vi "libssh2_userauth_publickey_fromfile_ex.vi"(5 "private key":path, 7 "public key":path, 8 "error in (no error)":errorcluster, 9 "passphrase":string, 10 "username":string, 11 "session":T1) -> (0 "error out":errorcluster)   [LabVIEW 2017, in "libssh2.lvlib"]
doc: "Authenticate a session using a private and public key file."
uses:
  libssh2.lvlib
  Session Refnum.ctl
  Not A Session.vi
  <vilib>/Utility/error.llb/Error Cluster From Error Code.vi
  Global Settings.vi
  Read Session Refnum.vi
  <vilib>/Utility/semaphor.llb/Acquire Semaphore.vi
  <vilib>/Utility/semaphor.llb/Release Semaphore.vi
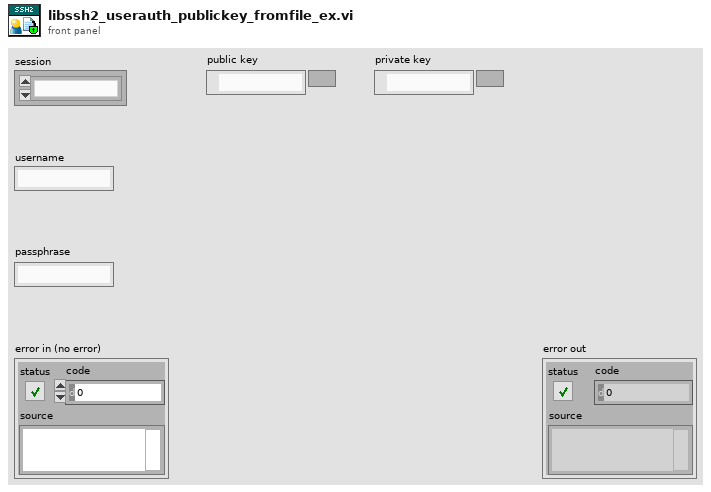
[diagram p1: front panel]
types:
  T1 = typedef "libssh2.lvlib/Session Refnum.ctl" = refnum<k1>
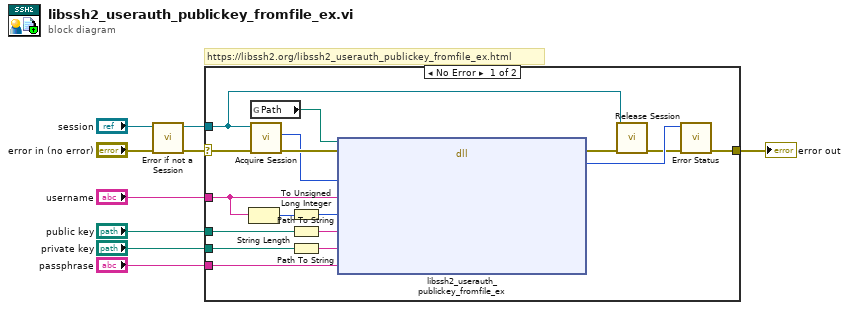
[diagram p0: block diagram]
diagram:
  # "https://libssh2.org/libssh2_userauth_publickey_fromfile_ex.html"
  n1 = call "Error if not a Session.vi"("error in (no error)"="error in (no error)", "session"="session") -> ("error out"=w6:errorcluster, "session out"=w4:T1)  [unwired: 8 in]
  n2 = case shown="No Error" w6 {
    selector: w6 -> [w25 w27]
    tunnel: "username" -> [w26 _]
    tunnel: [w24 w27] -> w8
    tunnel: w4 -> [w10 _]
    tunnel: "public key" -> [w16 _]
    tunnel: "private key" -> [w15 _]
    tunnel: "passphrase" -> [w14 _]
    frame No Error {
      n3 = String Length(string=w26) -> (length=w21:i32)
      n4 = global read "Global Settings.vi" "Path"() -> (w18:path)
      n5 = call "Acquire Session.vi"("error in (no error)"=w25, "session"=w10) -> ("error out"=w20:errorcluster, "LIBSSH2_SESSION*"=w19:u64)  [unwired: 7 in, 1 out]
      n6 = To Unsigned Long Integer(number=w21) -> (unsigned 32bit integer=w23:u32)
      n7 = Path To String(path=w16) -> (string=w13:string)
      n8 = Path To String(path=w15) -> (string=w12:string)
      n9 = dll-call lib="?" fn="libssh2_userauth_publickey_fromfile_ex"(path in=w18, error in=w20, "session"=w19, "username"=w26, "username_len"=w23, "publickey"=w13, "privatekey"=w12, "passphrase"=w14) -> (error out=w22:errorcluster, "return value"=w17:i32)  [unwired: 7 in, 1 out]
      n10 = call "Release Session.vi"("error in (no error)"=w22, "session"=w10) -> ("error out"=w11:errorcluster)  [unwired: 9 in]
      n11 = call "Error Status.vi"("error in (no error)"=w11, "return value"=w17) -> ("error out"=w24:errorcluster)  [unwired: 8 in, 1 out]
    }
    frame Error {
    }
  }
  "error out" <- w8
